vi "[ce] CalcExpress - Parse Script.vi"(5 "directives":T1={"enaNamedConst"=TRUE}, 6 "error in":errorcluster, 7 "create instance":bool, 8 "load FuncVIs":u32(ring)=2 items=["don't load", "load", "load & test"], 9 "expression":string) -> (0 "error out":errorcluster, 1 "new instance":bool, 2 "loaded functions":string[](array[string]), 3 "CE InstanceRef":T2)   [LabVIEW 2021]
doc: "This VI parses CalcExpress expressions and sequential scripts. A parsed script can be executed using a CalcExpress evaluator VI. To process non-sequential scripts that contain loops and conditional branching, use <b>CSE VIs</b>. Refer to the VI help for more details.\n\n<b>expression</b> specifies the CalcExpress expression or sequential script to be parsed.\n\n<b>load FuncVIs</b> control specifies how this VI maintains calls to FuncVI functions found during parsing:\n 'don't load' : does not load FuncVIs.\n 'load' : loads FuncVIs.\n 'load & test' : loads FuncVIs and verifies the correct number of arguments in the function calls.\n\n<b>create instance</b> control, if TRUE, causes the VI to create a new dynamic CalcExpress instance context. Every dynamic CalcExpress instance context must be explicitly closed using <b>[ce] CalcExpress - Close Instance.vi</b>.\n\n<b>CE InstanceRef</b> indicator returns a reference to a CalcExpress instance context containing the parsed expression.\n\n<b>new instance</b> indicator returns TRUE if a dynamic CalcExpress instance context has been created.\n\n::: CalcExpress Toolkit :::\nCopyright (c) 2000-2026 Konstantin Shifershteyn. All rights reserved."
uses:
  cetypes.llb/CalcExpress Instance RefNum.ctl
  cetypes.llb/CalcExpress Parsing Directives.ctl
  cersrc/celveng32.dll
panel:
  in  "CE InstanceRef Tmpl":T2
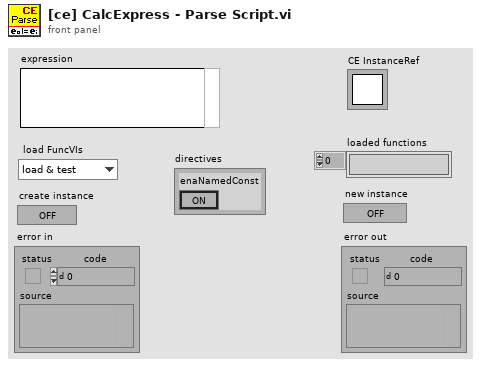
[diagram p1: front panel]
types:
  T1 = typedef "CalcExpress Parsing Directives.ctl" = cluster{"enaNamedConst":bool}
  T2 = typedef "CalcExpress Instance RefNum.ctl" = refnum<k1>
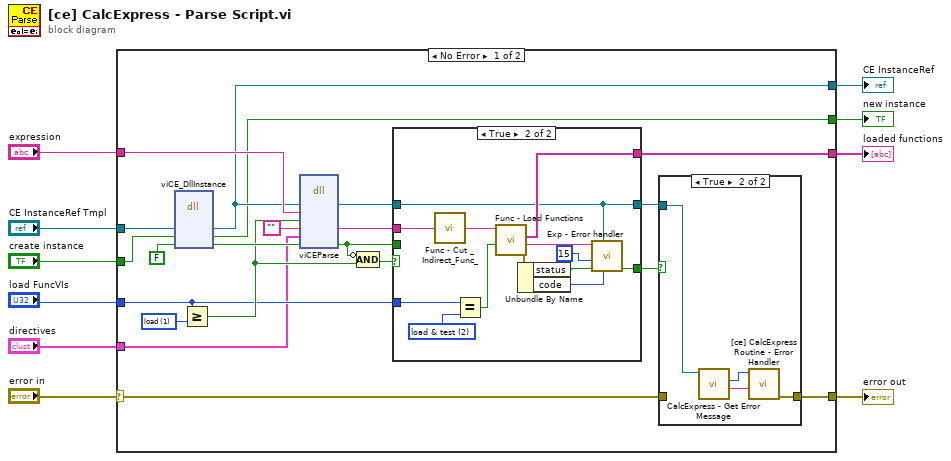
[diagram p0: block diagram]
diagram:
  n1 = case shown="No Error" "error in" {
    selector: "error in" -> [w12 w52]
    tunnel: [w25 w52] -> w10
    tunnel: "load FuncVIs" -> [w23 _]
    tunnel: "expression" -> [w21 _]
    tunnel: "create instance" -> [w20 _]
    tunnel: "CE InstanceRef Tmpl" -> [w19 _]
    tunnel: [w18 _] -> w5
    tunnel: [w17 _] -> w4
    tunnel: [w16 _] -> w3
    tunnel: "directives" -> [w14 _]
    frame No Error {
      w22 = u32 1 items=["don't load", "load", "load & test"] ("load FuncVIs")
      n2 = dll-call lib="C:/LV Projects/CalcExpress 40 LV2021/vi.lib/addons/CalcExpress/cersrc/celveng*.dll" fn="viCE_DllInstance"("iRef"=w19, "newInst"=w20, FALSE) -> ("iRef"=w17:T2, "newInst"=w16:bool, w29:bool)  [unwired: 6 in, 2 out]
      n3 = Greater Or Equal?(x=w23, y=w22) -> (x >= y?=w27:bool)
      n4 = dll-call lib="C:/LV Projects/CalcExpress 40 LV2021/vi.lib/addons/CalcExpress/cersrc/celveng*.dll" fn="viCEParse"("iRef"=w17, "script"=w21, "fFVI"=w27, "sFVI"="", "dirs"=w14, "erf"=w29) -> ("iRef"=w31:T2, "sFVI"=w30:string, "erf"=w15:bool)  [unwired: 7 in, 2 out]
      n5 = Compound Arithmetic op=AND(invert w15, w27) -> (w26:bool)
      n6 = case shown="True" w26 {
        tunnel: w31 -> [w32 w38]
        tunnel: [w33 w46] -> w11
        tunnel: w30 -> [_ w34]
        tunnel: [_ w45] -> w18
        tunnel: w15 -> [w33 _]
        tunnel: w23 -> [_ w41]
        tunnel: [w32 w38] -> w24
        frame False {
        }
        frame True {
          w40 = u32 2 items=["don't load", "load", "load & test"] ("load FuncVIs")
          n7 = call "Func - Cut _Indirect_Func_.vi"("FuncVI List"=w34) -> ("FuncVI List out"=w35:string)  [unwired: 4 in]
          n8 = Equal?(x=w41, y=w40) -> (x = y?=w39:bool)
          n9 = call "Func - Load Functions.vi"("test arg num (F)"=w39, "List of func names"=w35) -> ("error out"=w43:errorcluster, "error message"=w44:string, "loaded functions"=w45:string[])  [unwired: 5 in]
          n10 = Unbundle By Name(w43) -> ("status"=w42:bool, "code"=w36:i32)
          n11 = call "Exp - Error handler.vi"("error code in"=w36, "InstanceRef"=w38, "error in"=w42, "cmd (1:set)"=15, "error message in"=w44) -> ("error out"=w46:bool)  [unwired: 4 in, 2 out]
        }
      }
      n12 = case shown="True" w11 {
        tunnel: w12 -> [w47 _]
        tunnel: [w47 w51] -> w25
        tunnel: w24 -> [_ w49]
        frame False {
        }
        frame True {
          n13 = call "CalcExpress - Get Error Message.vi"("CE InstanceRef"=w49) -> ("error description"=w50:string, "error code"=w48:i32)  [unwired: 5 in, 2 out]
          n14 = call "[ce] CalcExpress Routine - Error Handler.vi"("error msg"=w50, "error code"=w48) -> ("error out"=w51:errorcluster)  [unwired: 7 in]
        }
      }
    }
    frame Error {
    }
  }
  "error out" <- w10
  "CE InstanceRef" <- w4
  "new instance" <- w3
  "loaded functions" <- w5
